vi "SimpleGit-LeaveDailyBranch.vi"(11 "path":path) -> (3 "f":string)   [LabVIEW 2017]
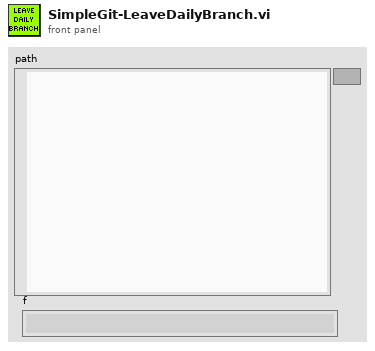
[diagram p1: front panel]
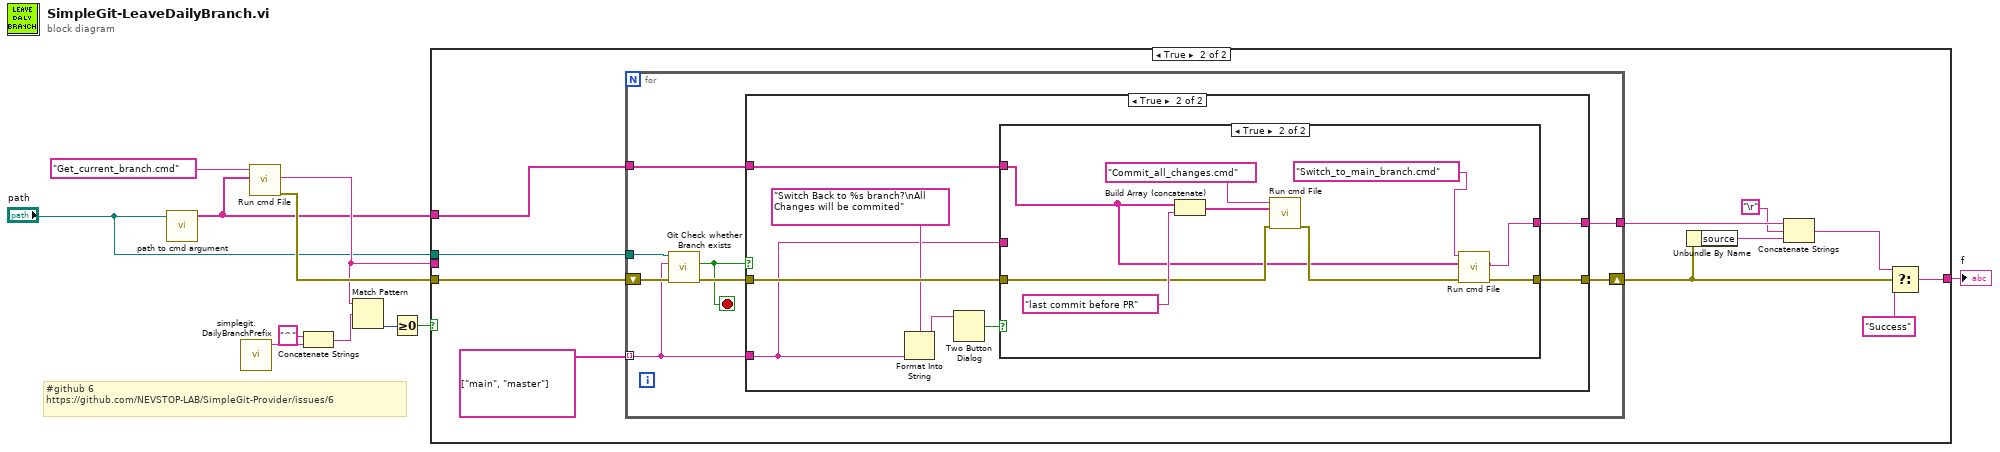
[diagram p0: block diagram]
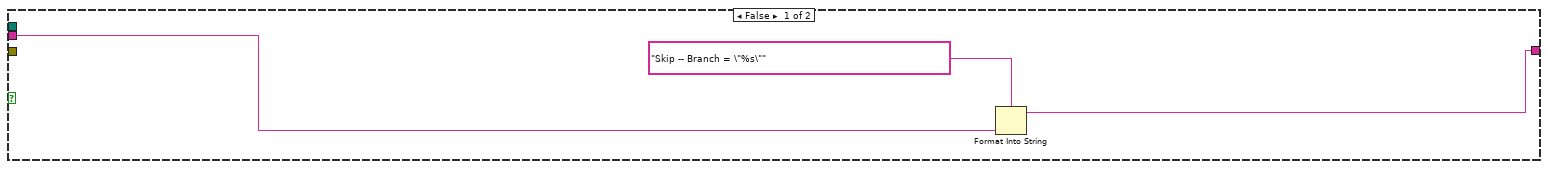
[diagram p2: hidden frame]
diagram:
  # "#github 6\nhttps://github.com/NEVSTOP-LAB/SimpleGit-Provider/issues/6"
  n1 = call "path to cmd argument.vi"("path"="path") -> ("Array"=w2:string[])  [unwired: 10 in]
  n2 = call "simplegit.DailyBranchPrefix.vi"() -> ("value"=w8:string)  [unwired: 11 in]
  n3 = call "Run cmd File.vi"("args"=w2, "name or relative path"="Get_current_branch.cmd") -> ("Error out"=w4:errorcluster, "before substring"=w3:string)  [unwired: 7 in, 1 out]
  n4 = Concatenate Strings("^" ("string"), w8) -> (w6:string)
  n5 = Match Pattern(string=w3, regular expression=w6) -> (offset past match=w10:i32)  [unwired: 1 in, 3 out]
  n6 = Greater Or Equal To 0?(x=w10) -> (x >= 0?=w11:bool)
  n7 = case shown="True" w11 {
    tunnel: w4 -> [_ w17]
    tunnel: w3 -> [w14 _]
    tunnel: [w12 w19] -> w9
    tunnel: w2 -> [_ w16]
    tunnel: "path" -> [_ w15]
    frame False {
      n8 = Format Into String(format string="Skip -- Branch = \"%s\"" ("f"), w14) -> (resulting string=w12:string)  [unwired: 2 in, 1 out]
    }
    frame True {
      n9 = for {
        tunnel: [w33] -> w23
        shift-right: [w32] -> w21
        shift-left: w17 -> [w31]
        tunnel: string[] ["main", "master"] ("x") -> [w28] mode=indexing
        tunnel: w16 -> [w27]
        tunnel: w15 -> [w26]
        stop <- w29 stop-if-true
        n10 = call "Git Check whether Branch exists.vi"("error in (no error)"=w31, "DailyPatchBranchName"=w28, "Path"=w26) -> ("error out"=w30:errorcluster, "Boolean"=w29:bool)  [unwired: 7 in]
        n11 = case shown="True" w29 {
          tunnel: [_ w41] -> w33
          tunnel: [w34 w40] -> w32
          tunnel: w30 -> [w34 w39]
          tunnel: w28 -> [_ w37]
          tunnel: w27 -> [_ w35]
          frame False {
          }
          frame True {
            n12 = Format Into String(format string="Switch Back to %s branch?\nAll Changes will be commited" ("message"), w37) -> (resulting string=w36:string)  [unwired: 2 in, 1 out]
            n13 = Two Button Dialog(message=w36) -> (T button?=w42:bool)  [unwired: 2 in]
            n14 = case shown="True" w42 {
              tunnel: [w43 w47] -> w40
              tunnel: [_ w46] -> w41
              tunnel: w39 -> [w43 w49]
              tunnel: w37 -> [_ _]
              tunnel: w35 -> [_ w44]
              frame False {
              }
              frame True {
                n15 = Build Array (concatenate)(w44, "last commit before PR" ("msg")) -> (w50:string[])
                n16 = call "Run cmd File.vi"("Error in"=w49, "args"=w50, "name or relative path"="Commit_all_changes.cmd") -> ("Error out"=w48:errorcluster)  [unwired: 6 in, 2 out]
                n17 = call "Run cmd File.vi"("Error in"=w48, "args"=w44, "name or relative path"="Switch_to_main_branch.cmd") -> ("Error out"=w47:errorcluster, "before substring"=w46:string)  [unwired: 6 in, 1 out]
              }
            }
          }
        }
      }
      n18 = Unbundle By Name(w21) -> ("source"=w24:string)
      n19 = Concatenate Strings(w23, "\r", w24) -> (w25:string)
      n20 = Select(t=w25, s=w21, f="Success") -> (s? t:f=w19:string)
    }
  }
  "f" <- w9
